vi "ReadDOs.vi"(7 "GroveConnector":enum16{"D16", "D18", "D20"}(ring), 8 "error in (no error)":errorcluster, 11 "Session in":refnum<class "Session.lvclass">) -> (0 "error out":errorcluster, 1 "DO 2 Status":bool, 2 "DO 1 Status":bool, 3 "Session out":refnum<class "Session.lvclass">)   [LabVIEW 2020]
uses:
  CTI/Session/Session.lvclass
  CTI/GPIO Direction.ctl
  CTI/GPIO Number.ctl
  CTI/CTI.lvlib
panel:
  # "Input"
  # "Output"
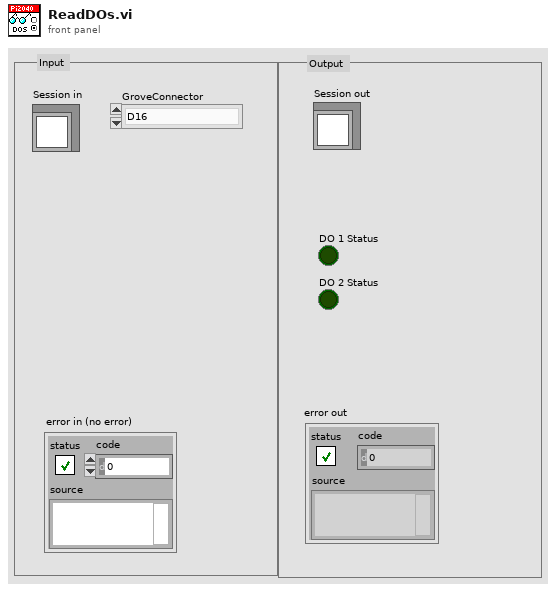
[diagram p1: front panel]
types:
  T1 = typedef "CTI.lvlib/GPIO Direction.ctl" = enum16{"In", "Out"}
  T2 = typedef "CTI.lvlib/GPIO Number.ctl" = i8
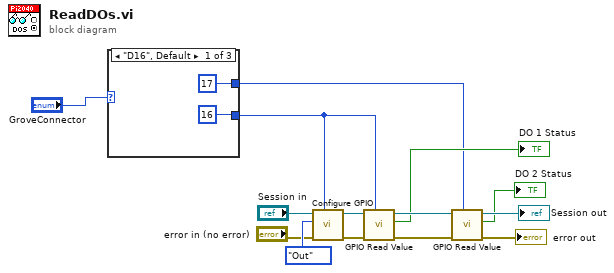
[diagram p0: block diagram]
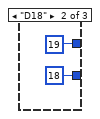
[diagram p2: hidden frame]
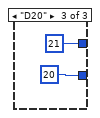
[diagram p3: hidden frame]
diagram:
  n1 = case shown="\"D16\", Default" "GroveConnector" {
    tunnel: [T2 16 ("GPIO #") T2 18 ("GPIO #") T2 20 ("GPIO #")] -> w4
    tunnel: [T2 17 ("GPIO #") T2 19 ("GPIO #") T2 21 ("GPIO #")] -> w1
    frame "D16", Default {
    }
    frame "D18" {
    }
    frame "D20" {
    }
  }
  n2 = call "Configure GPIO.vi"("GPIO #"=w4, "error in (no error)"="error in (no error)", "GPIO Direction"=GPIO_Direction."Out", "Session in"="Session in") -> ("error out"=w7:errorcluster, "Session out"=w8:refnum<class "Session.lvclass">)  [unwired: 6 in]
  n3 = call "GPIO Read Value.vi"("GPIO #"=w4, "error in (no error)"=w7, "Session in"=w8) -> ("error out"=w6:errorcluster, "Value"=→"DO 1 Status":bool, "Session out"=w5:refnum<class "Session.lvclass">)  [unwired: 6 in]
  n4 = call "GPIO Read Value.vi"("GPIO #"=w1, "error in (no error)"=w6, "Session in"=w5) -> ("error out"=→"error out":errorcluster, "Value"=→"DO 2 Status":bool, "Session out"=→"Session out":refnum<class "Session.lvclass">)  [unwired: 6 in]
